vi "Create.vi"(7 "Size":i32, 8 "error in (no error)":errorcluster, 10 "Group Config":refnum<class "Group Config.lvclass">) -> (0 "error out":errorcluster, 3 "Group Buffer DBL out":refnum<class "Group Buffer DBL.lvclass">)   [LabVIEW 2020, in "VolatusHistorian.lvlib" / "Group Buffer DBL.lvclass"]
uses:
  Group Buffer DBL.lvclass
  VolatusConfig/Group/Group Config.lvclass
  Ref.ctl
  lv-vecto/Vecto/Group Info.ctl
  Channel Buffer DBL/Channel Buffer DBL.lvclass
  Group Buffer DBL.lvclass/Group Buffer DBL.ctl
  lv-vecto/Vecto/Group Config/Group Config.lvclass
  VolatusConfig/Channel/Channel Config.lvclass
  lv-vecto/VectoConfig/VectoConfig.lvlib
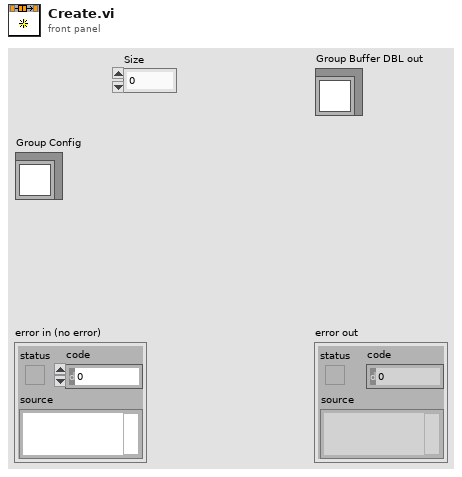
[diagram p1: front panel]
types:
  T1 = typedef "VolatusHistorian.lvlib/Group Buffer DBL.lvclass/Ref.ctl" = cluster{"Time":refnum<queue>, "Channel Name Map":map{string, i32}, "Group Info":T2, "Channels":refnum<class "Channel Buffer DBL.lvclass">[], "Channel Names":string[]}
  T2 = typedef "VectoConfig.lvlib/Group Info.ctl" = cluster{"System":string, "Cluster":string, "Node":string, "Task":string, "Name":string}
  T3 = typedef "VectoConfig.lvlib/Channel Info.ctl" = cluster{"Name":string, "Group":string, "Owning Node":string, "Owning Task":string, "Resource":string}
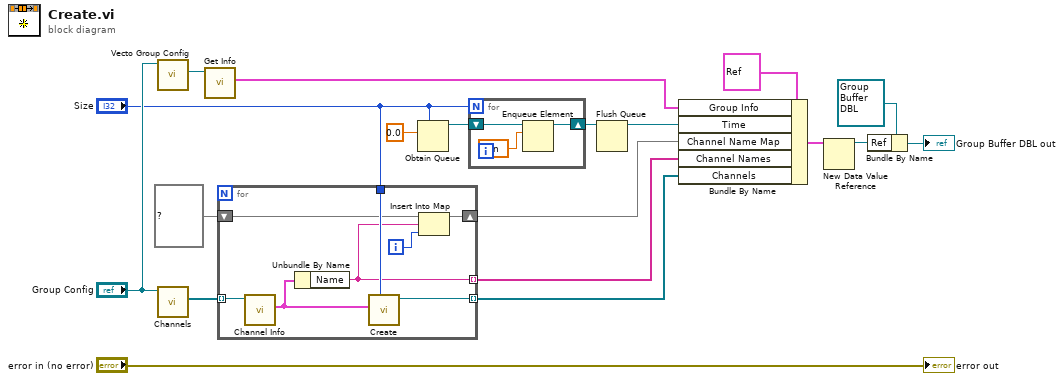
[diagram p0: block diagram]
diagram:
  n1 = call "Vecto Group Config.vi"("Group in"="Group Config") -> ("Vecto Group Config"=w19:refnum<class "Group Config.lvclass">)  [unwired: 8 in, 2 out]
  n2 = call "Channels.vi"("Group in"="Group Config") -> ("Channels"=w15:refnum<class "Channel Config.lvclass">[])  [unwired: 8 in, 2 out]
  n3 = call "Get Info.vi"("Group Config in"=w19) -> ("Info"=w18:T2)  [unwired: 8 in, 2 out]
  n4 = for {
    tunnel: w15 -> [w27] mode=indexing
    shift-right: [w23] -> w13
    shift-left: map{string, i32} {} ("Channels") -> [w24]
    tunnel: "Size" -> [w26]
    tunnel: [w22] -> w11 mode=indexing
    tunnel: [w20] -> w10 mode=indexing
    i -> [w21]
    n5 = call "Channel Info.vi"("Channel in"=w27) -> ("Channel Info"=w25:T3)  [unwired: 8 in, 2 out]
    n6 = Unbundle By Name(w25) -> ("Name"=w20:string)
    n7 = call "Create.vi"("Size"=w26, "Channel Info"=w25) -> ("Channel Buffer DBL out"=w22:refnum<class "Channel Buffer DBL.lvclass">)  [unwired: 8 in, 1 out]
    n8 = Insert Into Map(map in=w24, key=w20, value=w21) -> (map out=w23:map{string, i32})  [unwired: 2 out]
  }
  n9 = Obtain Queue(max queue size (-1, unlimited)="Size", element data type=0.0) -> (queue out=w3:refnum<queue>)  [unwired: 3 in, 2 out]
  n10 = for {
    N: "Size" -> [_]
    shift-right: [w28] -> w4
    shift-left: w3 -> [w30]
    n11 = Enqueue Element(queue=w30, element=nan) -> (queue out=w28:refnum<queue>)  [unwired: 2 in, 2 out]
  }
  n12 = Flush Queue(queue=w4) -> (queue out=w2:refnum<queue>)  [unwired: 1 in, 2 out]
  n13 = Bundle By Name(cluster=T1 {"Time"=refnum, "Channel Name Map"={}, "Group Info"={"System"="", "Cluster"="", "Node"="", "Task"="", "Name"=""}, "Channels"=[], "Channel Names"=[]} ("Ref"), "Group Info"=w18, "Time"=w2, "Channel Name Map"=w13, "Channel Names"=w10, "Channels"=w11) -> (w8:T1)
  n14 = New Data Value Reference(data value=w8) -> (data value reference=w6:refnum<data-value>)  [unwired: 1 in, 1 out]
  n15 = Bundle By Name(cluster=refnum<class "Group Buffer DBL.lvclass"> refnum ("Group Buffer DBL out"), "Ref"=w6) -> (→"Group Buffer DBL out":refnum<class "Group Buffer DBL.lvclass">)
  "error out" <- "error in (no error)"
